vi "SeqEditor_getConPanekids_GetNLTinfo.vi"(11 "reference in":refnum<vi>) -> (1 "typedata":string, 2 "CtrlTextValue":string, 3 "TYPE":T1=enum."VISA")   [LabVIEW 2017, in "NLTest.lvclass"]
uses:
  NLTest.lvclass
  VISTEP_class_INOUTPUT_TYPE.ctl
panel:
  out "TypeDataStrings[]":string[](array[string])
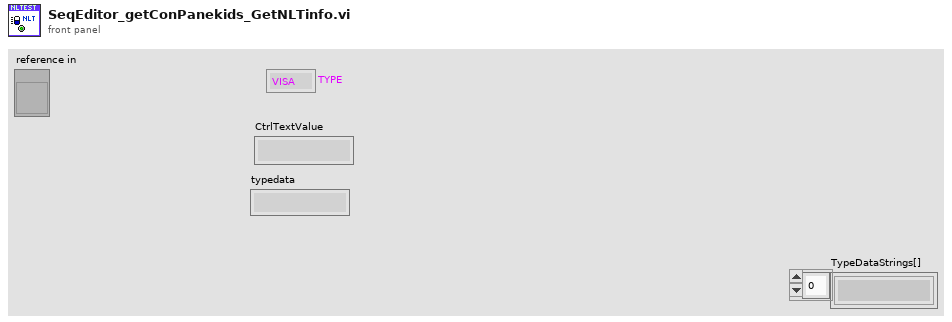
[diagram p1: front panel]
types:
  T1 = typedef "NLTest.lvclass/VISTEP_class_INOUTPUT_TYPE.ctl" = enum16{"Number", "String", "Bool", "Enum", "Path", "VISA", "NA"}
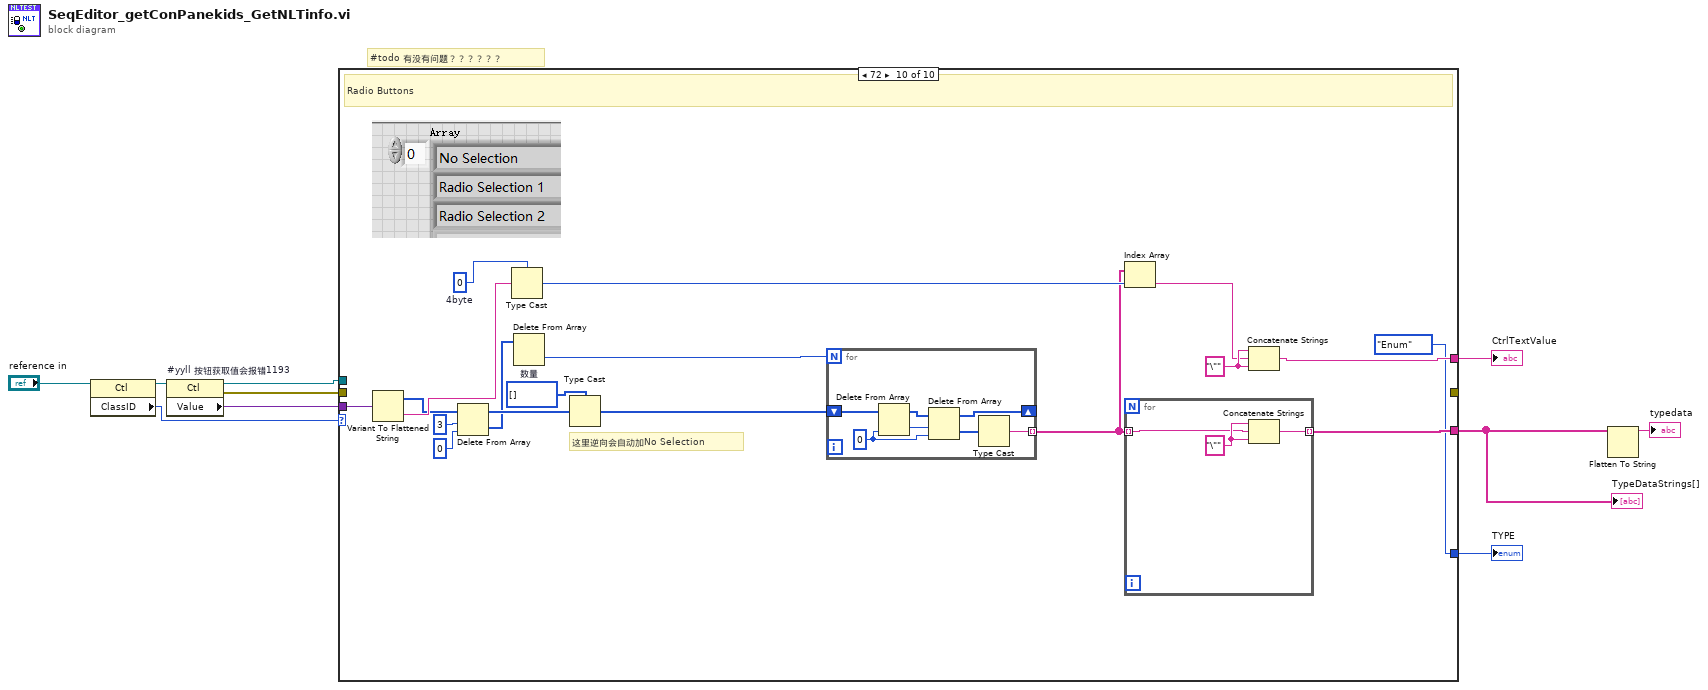
[diagram p0: block diagram]
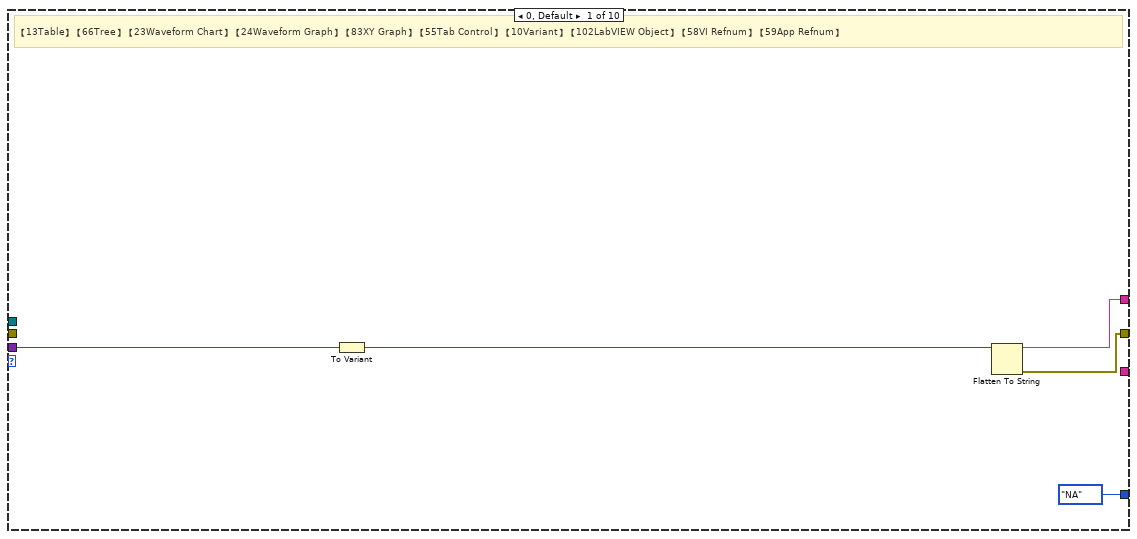
[diagram p2: hidden frame]
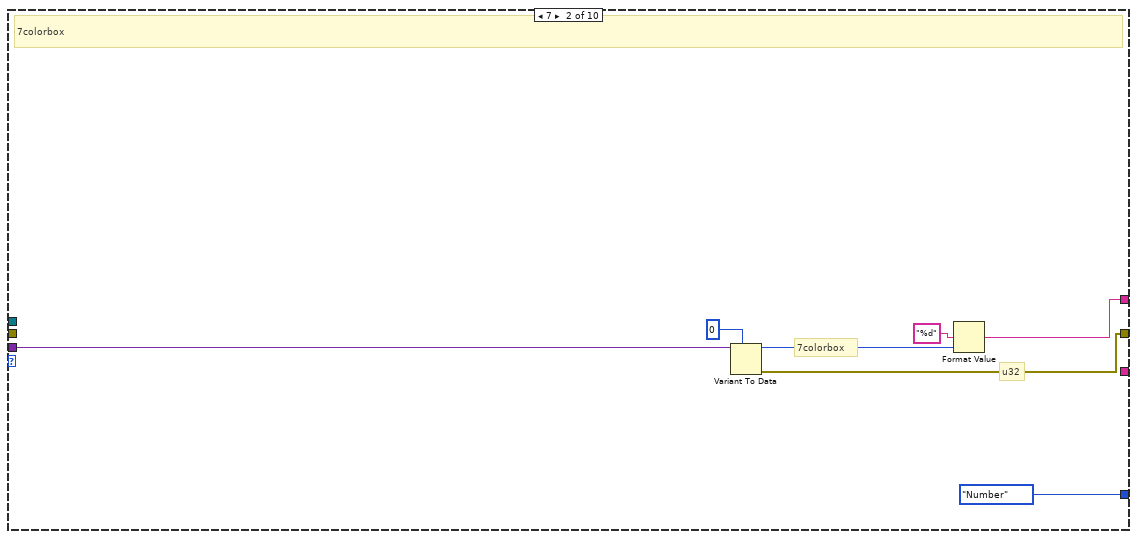
[diagram p3: hidden frame]
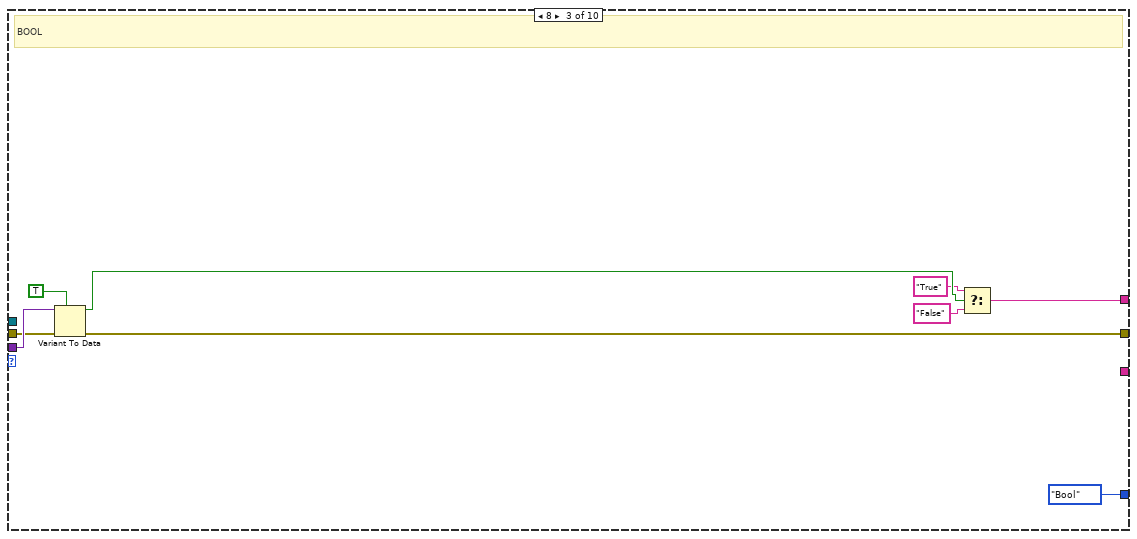
[diagram p4: hidden frame]
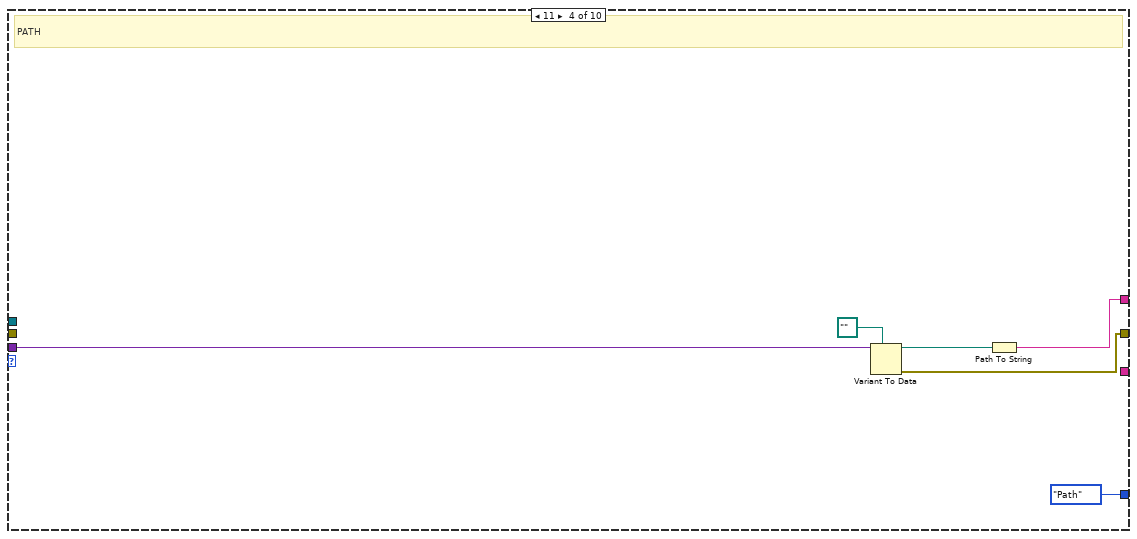
[diagram p5: hidden frame]
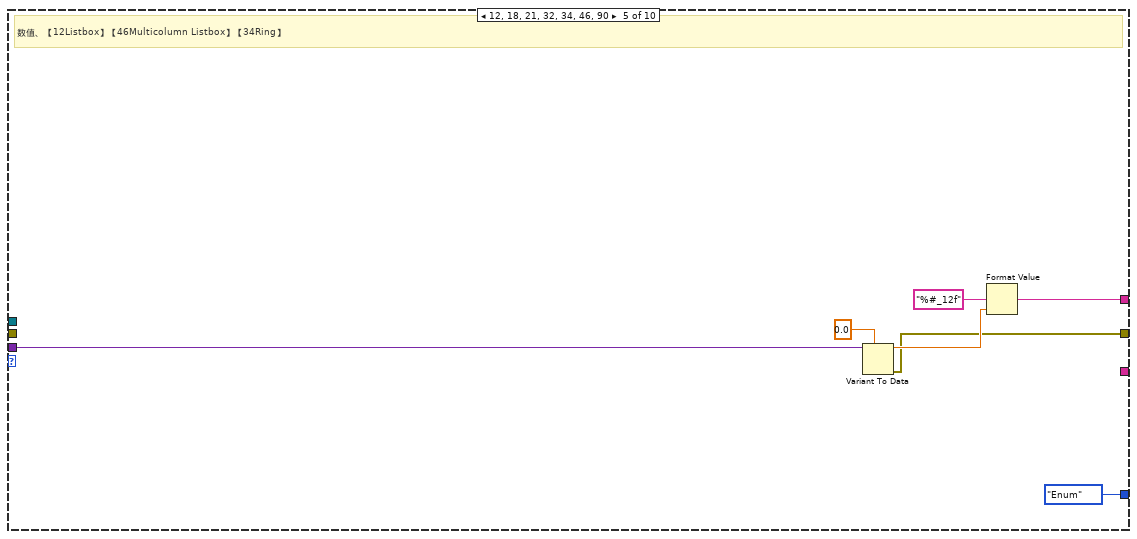
[diagram p6: hidden frame]
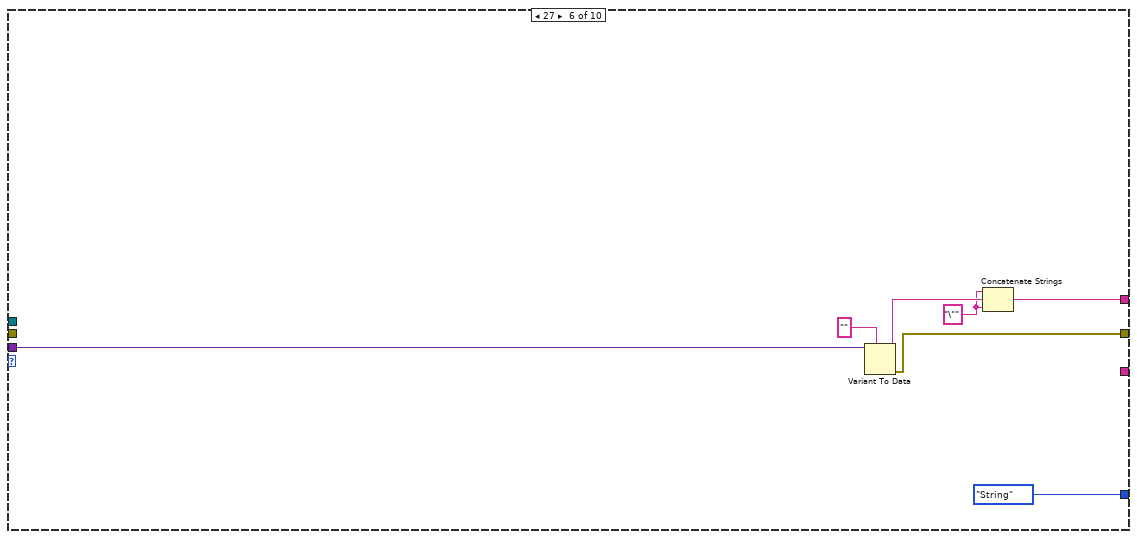
[diagram p7: hidden frame]
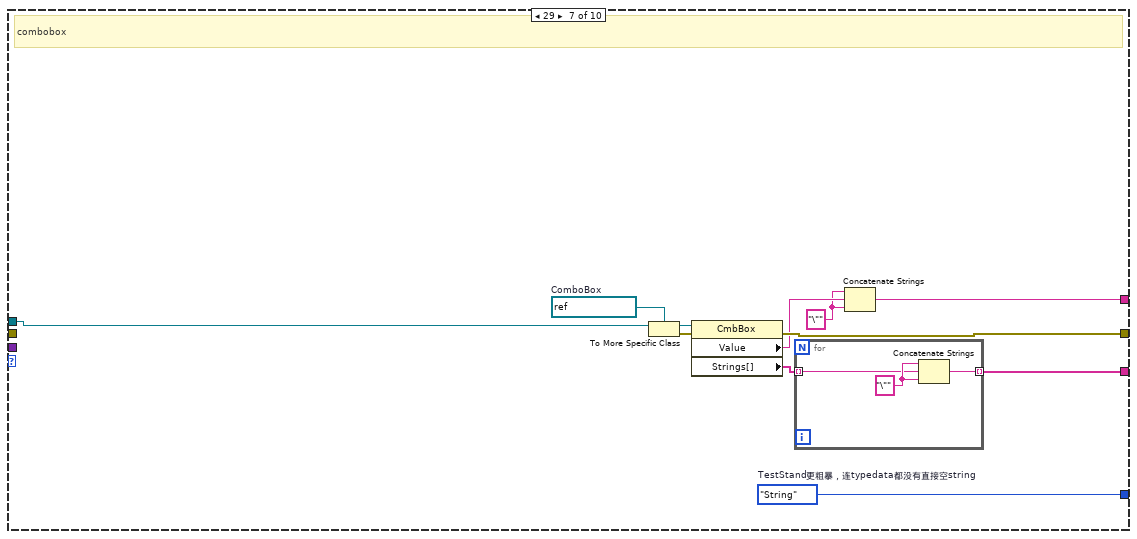
[diagram p8: hidden frame]
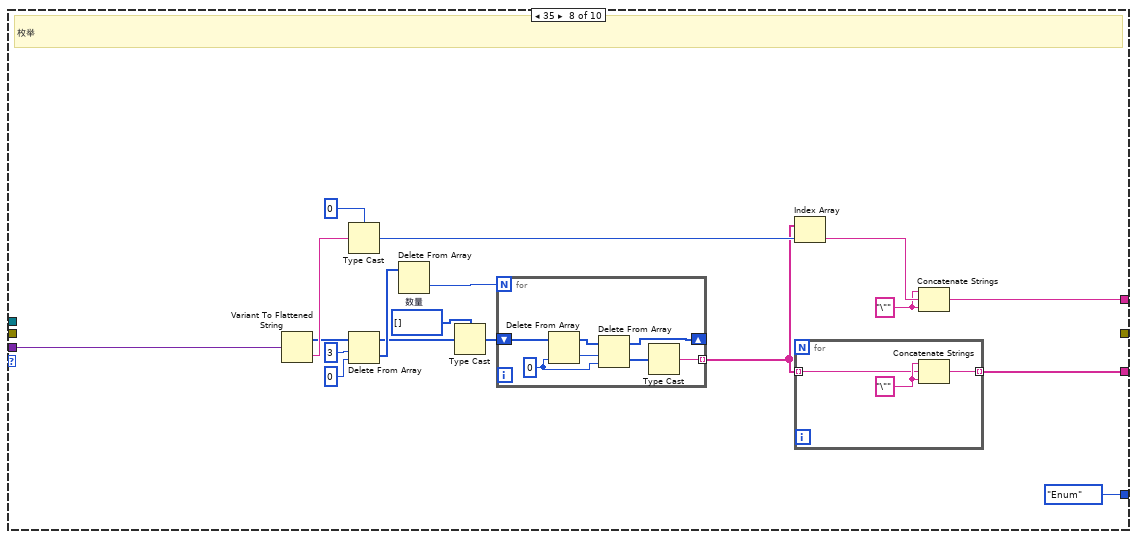
[diagram p9: hidden frame]
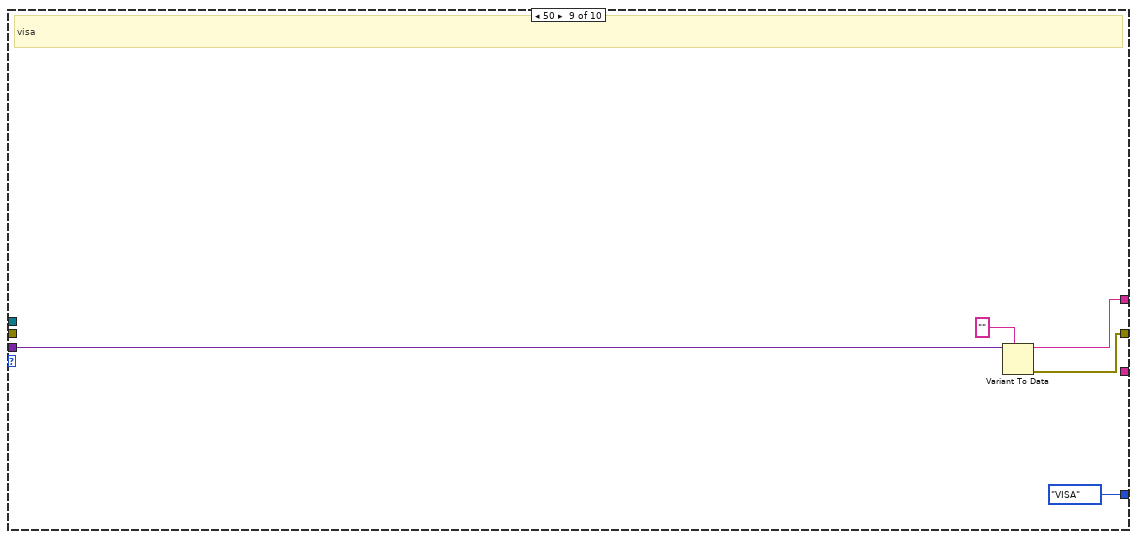
[diagram p10: hidden frame]
diagram:
  # "#todo 有没有问题？？？？？？"
  n1 = property class="Ctl"(reference="reference in") -> (reference out=w6:refnum<vi>, "ClassID"=w10:u32)  [unwired: 1 in, 1 out]
  n2 = property on="#yyll 按钮获取值会报错1193" class="Ctl"(reference=w6) -> (reference out=w7:refnum<vi>, error out=w4:errorcluster, "Value"=w5:variant)  [unwired: 1 in]
  n3 = case shown="72" w10 {
    tunnel: w5 -> [w13 w22 w31 w37 w44 w51 _ w83 w98 w114]
    tunnel: [w15 w18 w26 w33 w40 w47 w56 w70 w96 w107] -> w8
    tunnel: [w14 w17 w25 w35 w39 w48 w58 _ w95 _] -> _
    tunnel: w7 -> [_ _ _ _ _ _ w61 _ _ _]
    tunnel: [_ _ _ _ _ _ w53 w67 _ w109] -> w2
    tunnel: w4 -> [_ _ w24 _ _ _ _ _ _ _]
    tunnel: [VISTEP_class_INOUTPUT_TYPE."NA" ("TYPE") VISTEP_class_INOUTPUT_TYPE."Number" ("TYPE") VISTEP_class_INOUTPUT_TYPE."Bool" ("TYPE") VISTEP_class_INOUTPUT_TYPE."Path" ("TYPE") VISTEP_class_INOUTPUT_TYPE."Enum" ("TYPE") VISTEP_class_INOUTPUT_TYPE."String" ("TYPE") w52 VISTEP_class_INOUTPUT_TYPE."Enum" ("TYPE") VISTEP_class_INOUTPUT_TYPE."VISA" ("TYPE") VISTEP_class_INOUTPUT_TYPE."Enum" ("TYPE")] -> w3
    frame 0, Default {
      # "【13Table】【66Tree】【23Waveform Chart】【24Waveform Graph】【83XY Graph】【55Tab Control】【10Variant】【102LabVIEW Object】【58VI Refnum】【59App Refnum】"
      n4 = To Variant(anything=w13) -> (Variant=w12:variant)
      n5 = Flatten To String(anything=w12) -> (data string=w15:string, error out=w14:errorcluster)  [unwired: 3 in, 1 out]
    }
    frame 7 {
      # "u32"
      # "7colorbox"
      # "7colorbox"
      n6 = Variant To Data(type=u32 0, Variant=w22) -> (data=w20:u32, error out=w17:errorcluster)  [unwired: 1 in]
      n7 = Format Value(format string="%d", value (0)=w20) -> (output string=w18:string)  [unwired: 1 in]
    }
    frame 8 {
      # "BOOL"
      n8 = Variant To Data(error in=w24, type=TRUE, Variant=w31) -> (data=w29:bool, error out=w25:errorcluster)
      n9 = Select(t="True", s=w29, f="False") -> (s? t:f=w26:string)
    }
    frame 11 {
      # "PATH"
      n10 = Variant To Data(type=path "", Variant=w37) -> (data=w36:path, error out=w35:errorcluster)  [unwired: 1 in]
      n11 = Path To String(path=w36) -> (string=w33:string)
    }
    frame 12, 18, 21, 32, 34, 46, 90 {
      # "数值、【12Listbox】【46Multicolumn Listbox】【34Ring】"
      n12 = Variant To Data(type=0.0, Variant=w44) -> (data=w42:dbl, error out=w39:errorcluster)  [unwired: 1 in]
      n13 = Format Value(format string="%#_12f", value (0)=w42) -> (output string=w40:string)  [unwired: 1 in]
    }
    frame 27 {
      w46 = "\"" ("string")
      n14 = Variant To Data(type="", Variant=w51) -> (data=w49:string, error out=w48:errorcluster)  [unwired: 1 in]
      n15 = Concatenate Strings(w46, w49, w46) -> (w47:string)
    }
    frame 29 {
      w52 = VISTEP_class_INOUTPUT_TYPE."String"  # TestStand更粗暴，连typedata都没有直接空string
      w55 = "\"" ("string")
      w62 = refnum<vi> refnum  # ComboBox
      # "combobox"
      n16 = To More Specific Class(target class=w62, reference=w61) -> (specific class reference=w60:refnum<vi>, error out=w59:errorcluster)  [unwired: 1 in]
      n17 = property class="CmbBox"(reference=w60, error in=w59) -> (error out=w58:errorcluster, "Value"=w57:string, "Strings[]"=w54:string[])  [unwired: 1 out]
      n18 = for {
        tunnel: w54 -> [w64] mode=indexing
        tunnel: [w63] -> w53 mode=indexing
        w65 = "\"" ("string")
        n19 = Concatenate Strings(w65, w64, w65) -> (w63:string)
      }
      n20 = Concatenate Strings(w55, w57, w55) -> (w56:string)
    }
    frame 35 {
      w69 = "\"" ("string")
      # "枚举"
      n21 = Variant To Flattened String(Variant=w83) -> (data string=w81:string, 1:w80:i16[])
      n22 = Type Cast(type=u16 0 ("Numeric"), x=w81) -> (*(type *) &x=w71:u16)
      n23 = Delete From Array(array=w80, length=3, index=0) -> (deleted portion=w78:i16[], array with subset deleted=w74:i16[])
      n24 = Delete From Array "数量"(array=w78) -> (deleted portion=w76:i16)  [unwired: 2 in, 1 out]
      n25 = Type Cast(type=u8[] [], x=w74) -> (*(type *) &x=w73:u8[])
      n26 = for {
        N: w76 -> [_]
        shift-right: [w88] -> _
        shift-left: w73 -> [w93]
        tunnel: [w87] -> w68 mode=indexing
        w90 = 0 ("index")
        n27 = Delete From Array(array=w93, index=w90) -> (deleted portion=w91:u8, array with subset deleted=w92:u8[])  [unwired: 1 in]
        n28 = Delete From Array(array=w92, length=w91, index=w90) -> (deleted portion=w89:u8[], array with subset deleted=w88:u8[])
        n29 = Type Cast(x=w89) -> (*(type *) &x=w87:string)  [unwired: 1 in]
      }
      n30 = Index Array(array=w68, index=w71) -> (element=w82:string)
      n31 = for {
        tunnel: w68 -> [w85] mode=indexing
        tunnel: [w84] -> w67 mode=indexing
        w86 = "\"" ("string")
        n32 = Concatenate Strings(w86, w85, w86) -> (w84:string)
      }
      n33 = Concatenate Strings(w69, w82, w69) -> (w70:string)
    }
    frame 50 {
      # "visa"
      n34 = Variant To Data(type="", Variant=w98) -> (data=w96:string, error out=w95:errorcluster)  [unwired: 1 in]
    }
    frame 72 {
      w111 = "\"" ("string")
      w115 = 0  # 4byte
      # "这里逆向会自动加No Selection"
      # "Radio Buttons"
      n35 = Variant To Flattened String(Variant=w114) -> (data string=w116:string, 1:w112:i16[])
      n36 = Delete From Array(array=w112, length=3, index=0) -> (deleted portion=w103:i16[], array with subset deleted=w105:i16[])
      n37 = Type Cast(type=w115, x=w116) -> (*(type *) &x=w113:i32)
      n38 = Delete From Array "数量"(array=w103) -> (deleted portion=w104:i16)  [unwired: 2 in, 1 out]
      n39 = Type Cast(type=u8[] [], x=w105) -> (*(type *) &x=w106:u8[])
      n40 = for {
        N: w104 -> [_]
        shift-right: [w118] -> _
        shift-left: w106 -> [w123]
        tunnel: [w117] -> w110 mode=indexing
        w120 = 0 ("index")
        n41 = Delete From Array(array=w123, index=w120) -> (deleted portion=w121:u8, array with subset deleted=w122:u8[])  [unwired: 1 in]
        n42 = Delete From Array(array=w122, length=w121, index=w120) -> (deleted portion=w119:u8[], array with subset deleted=w118:u8[])
        n43 = Type Cast(x=w119) -> (*(type *) &x=w117:string)  [unwired: 1 in]
      }
      n44 = Index Array(array=w110, index=w113) -> (element=w108:string)
      n45 = for {
        tunnel: w110 -> [w125] mode=indexing
        tunnel: [w124] -> w109 mode=indexing
        w126 = "\"" ("string")
        n46 = Concatenate Strings(w126, w125, w126) -> (w124:string)
      }
      n47 = Concatenate Strings(w111, w108, w111) -> (w107:string)
    }
  }
  "CtrlTextValue" <- w8
  "TypeDataStrings[]" <- w2
  "TYPE" <- w3
  n48 = Flatten To String(anything=w2) -> (data string=→"typedata":string)  [unwired: 3 in, 2 out]
